vi "build.relative.vi"(9 "Offset":timestamp format="%<%x %.3X>T", 10 "Time Unit":T1(ring), 11 "Time Series Name":string) -> (3 "Timestamp Metadata":refnum<class "timestampMetadata.lvclass">)   [LabVIEW 2020, in "ts.relative.lvclass"]
uses:
  ts.relative.lvclass
  ts.relative.lvclass/ts.relative.ctl
  timestampMetadata/timestampMetadata.lvclass
  C:/code/labview-client/lv_src/timestampType/timestampType.lvclass
  C:/code/labview-client/lv_src/Nominal Client/datasources/payload/payload.lvclass
  C:/code/labview-client/lv_src/ts.relative/ts.relative.lvclass
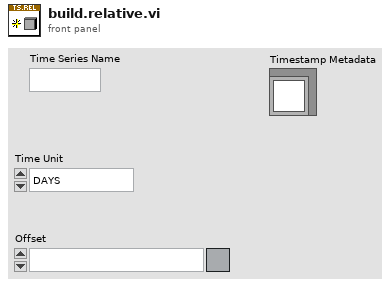
[diagram p1: front panel]
types:
  T1 = enum16{"DAYS", "HOURS", "MINUTES", "SECONDS", "MILLISECONDS", "MICROSECONDS", "NANOSECONDS", "PICOSECONDS"}
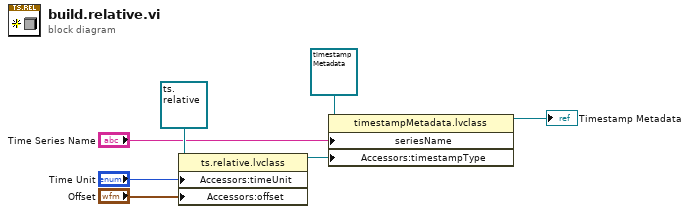
[diagram p0: block diagram]
diagram:
  n1 = property class="ts.relative.lvclass"(reference=refnum<class "ts.relative.lvclass"> refnum, "Accessors:timeUnit"="Time Unit", "Accessors:offset"="Offset") -> (reference out=w4:refnum<class "ts.relative.lvclass">)  [unwired: 1 in, 1 out]
  n2 = property class="timestampMetadata.lvclass"(reference=refnum<class "timestampMetadata.lvclass"> refnum ("timestampMetadata.lvclass"), "seriesName"="Time Series Name", "Accessors:timestampType"=w4) -> (reference out=→"Timestamp Metadata":refnum<class "timestampMetadata.lvclass">)  [unwired: 1 in, 1 out]
